vi "_MDPtr Unpack Memory.vi"(10 "error in (no error)":errorcluster, 11 "HexStrPtr":T1) -> (1 "String Attribute":string, 2 "error out":errorcluster, 3 "string":string)   [LabVIEW 2017, in "MDPtr.lvlib"]
uses:
  MDPtr.lvlib
  MDPtr TypeDef/MDPtr.ctl
  <vilib>/Utility/Data Type/Type Definitions/Data Type.ctl
  _MDPtrMgr/MDPtrMgr.lvclass
  <vilib>/Utility/Data Type/NI_Data Type.lvlib
panel:
  # "Connector Pane"
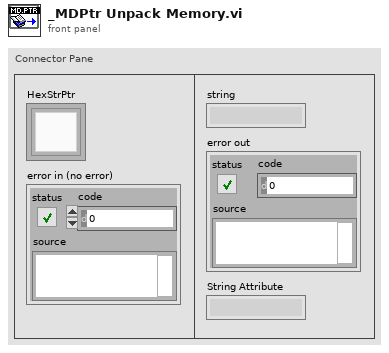
[diagram p1: front panel]
types:
  T1 = typedef "MDPtr.lvlib/MDPtr.ctl" = refnum<k1>
  T2 = typedef "NI_Data Type.lvlib/Data Type.ctl" = enum8{"Invalid Type", "Void", "I8", "I16", "I32", "I64", "U8", "U16", "U32", "U64", "Single Float", "Double Float", "Extended Float", "Single Complex", "Double Complex", "Extended Complex", "Enum U8", "Enum U16", "Enum U32", "Enum U64", "Single Float With Unit", "Double Float With Unit", "Extended Float With Unit", "Single Complex with Unit", "Double Complex with Unit", "Extended Complex with Unit", "Boolean", "String", "Path", "Picture", "Tag", "Array", "Cluster", "Variant", "LV Variant", "Waveform", "Timestamp", "Digital Waveform", "Digital Data", "ExpressData", "Refnum", "External Data", "VI", "Poly VI", "LabVIEW Class Instance", "Fixed Point"}
  T3 = typedef "MDPtr.lvlib/MDPtr DataFrame-Memory.ctl" = cluster{"Common":T4, "DVR":refnum<data-value>}
  T4 = typedef "MDPtr.lvlib/MDPtr DataFrame-Common.ctl" = cluster{"Data Type":T2, "Copy Count":i32, "String Attribute":string, "Cache Length":i32, "Data Length":i32}
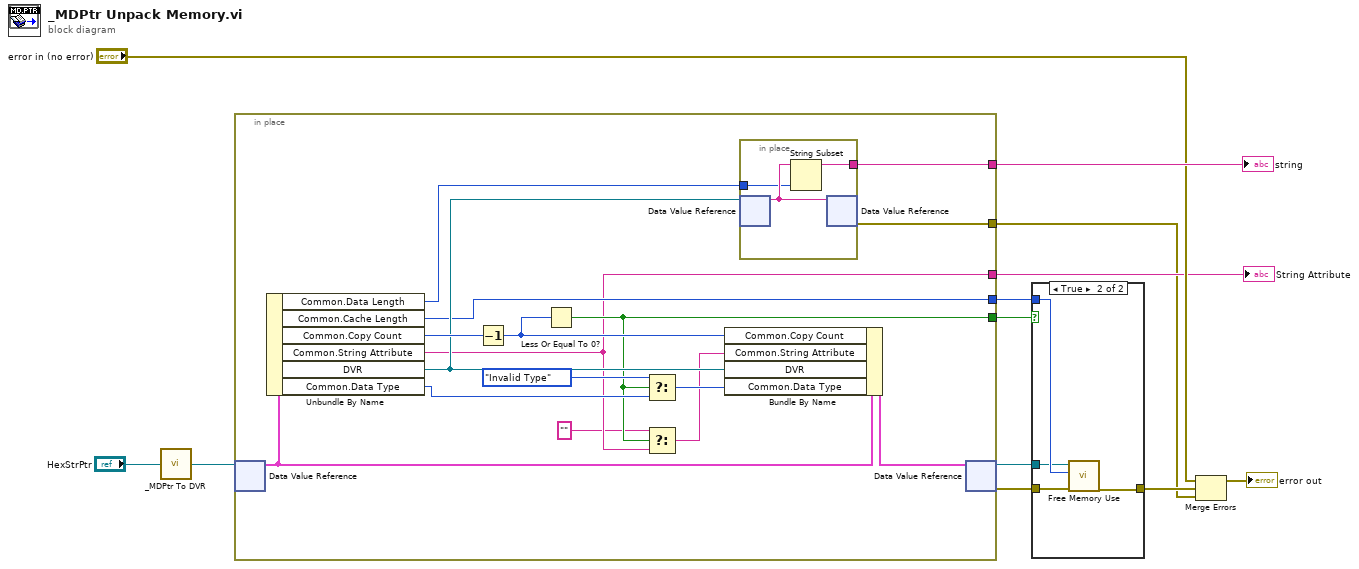
[diagram p0: block diagram]
diagram:
  n1 = call "_MDPtr To DVR.vi"("MDPtr"="HexStrPtr") -> ("MDPtr DVR"=w7:refnum<data-value>)
  n2 = in-place "In Place Element Structure" {
    in-place-border: [w25] -> w12
    in-place-border: [w15] -> w9
    in-place-border: [w16] -> w4
    in-place-border: [w21] -> w3
    in-place-border: [w20] -> w1
    n3 = in-place-dvr #1(w7) -> (w28:T3)  [unwired: 1 out]
    n4 = Unbundle By Name(w28) -> ("Common.Data Length"=w22:i32, "Common.Cache Length"=w21:i32, "Common.Copy Count"=w26:i32, "Common.String Attribute"=w15:string, "DVR"=w23:refnum<data-value>, "Common.Data Type"=w19:T2)
    n5 = Decrement(x=w26) -> (x-1=w24:i32)
    n6 = Less Or Equal To 0?(x=w24) -> (x <= 0?=w16:bool)
    n7 = Select(t=Data_Type."Invalid Type", s=w16, f=w19) -> (s? t:f=w17:T2)
    n8 = Select(t="", s=w16, f=w15) -> (s? t:f=w13:string)
    n9 = Bundle By Name(cluster=w28, "Common.Copy Count"=w24, "Common.String Attribute"=w13, "DVR"=w23, "Common.Data Type"=w17) -> (w27:T3)
    n10 = in-place {
      in-place-border: [w30] -> w25
      in-place-border: w22 -> [w29]
      n11 = in-place-dvr #2(w23) -> (w31:string)  [unwired: 1 out]
      n12 = String Subset(string=w31, length (rest)=w29) -> (substring=w30:string)  [unwired: 1 in]
      n13 = in-place-dvr #2(w31) -> (w20:errorcluster)  [unwired: 1 out]
    }
    n14 = in-place-dvr #1(w27) -> (w2:refnum<data-value>, w6:errorcluster)
  }
  "string" <- w12
  "String Attribute" <- w9
  n15 = case shown="True" w4 {
    tunnel: [_ w35] -> w5
    tunnel: w6 -> [_ w34]
    tunnel: w3 -> [_ w33]
    tunnel: w2 -> [_ w32]
    frame False {
    }
    frame True {
      n16 = call "Free Memory Use.vi"("error in"=w34, "Cache Length"=w33, "MDPtr DVR"=w32) -> ("error out"=w35:errorcluster)  [unwired: 8 in]
    }
  }
  n17 = Merge Errors("error in (no error)", w5, w1) -> (→"error out":errorcluster)
